vi "UnscentedKalmanFilter_SetXHat.vi"(10 "xHat":T1, 11 "in UnscentedKalmanFiilter":T2) -> (0 "SizeCoerced":bool, 3 "out UnscentedKalmanFiilter":T2)   [LabVIEW 2019, in "Trajectory_Library.lvlib"]
doc: "Set initial state estimate x-hat.\n \nInputs:\n - inUnscentedKalmanFilter -- filter data cluster\n - xHat -- The state estimate x-hat.\n\nOutputs:\n - outUnscentedKalmanFilter -- updated filter data cluster\n - sizeCoerced -- If TRUE, an error occured"
uses:
  Trajectory_Library.lvlib
  <vilib>/Analysis/Matrix/Datatypes/RealMatrix.ctl
  <vilib>/Analysis/Matrix/NI_Matrix.lvlib
  TypeDef/MERWE_SCALED_SIGMA_PTS.ctl
  TypeDef/UNSCENTED_KALMAN_FILTER.ctl
  TypeDef/CALLBACK_FUNC_TYPE.ctl
panel:
  # "State Estimate <Statess,1>"
  # "<States, States>"
  # "<States, ?>"
  # "<Statess,  States>"
  # "<Outputs, Outputs>"
  # "<?, 1>"
  # "<?, 1>"
  # "State Estimate <Statess,1>"
  # "<States, States>"
  # "<States, ?>"
  # "<Statess,  States>"
  # "<Outputs, Outputs>"
  # "<?, 1>"
  # "<?, 1>"
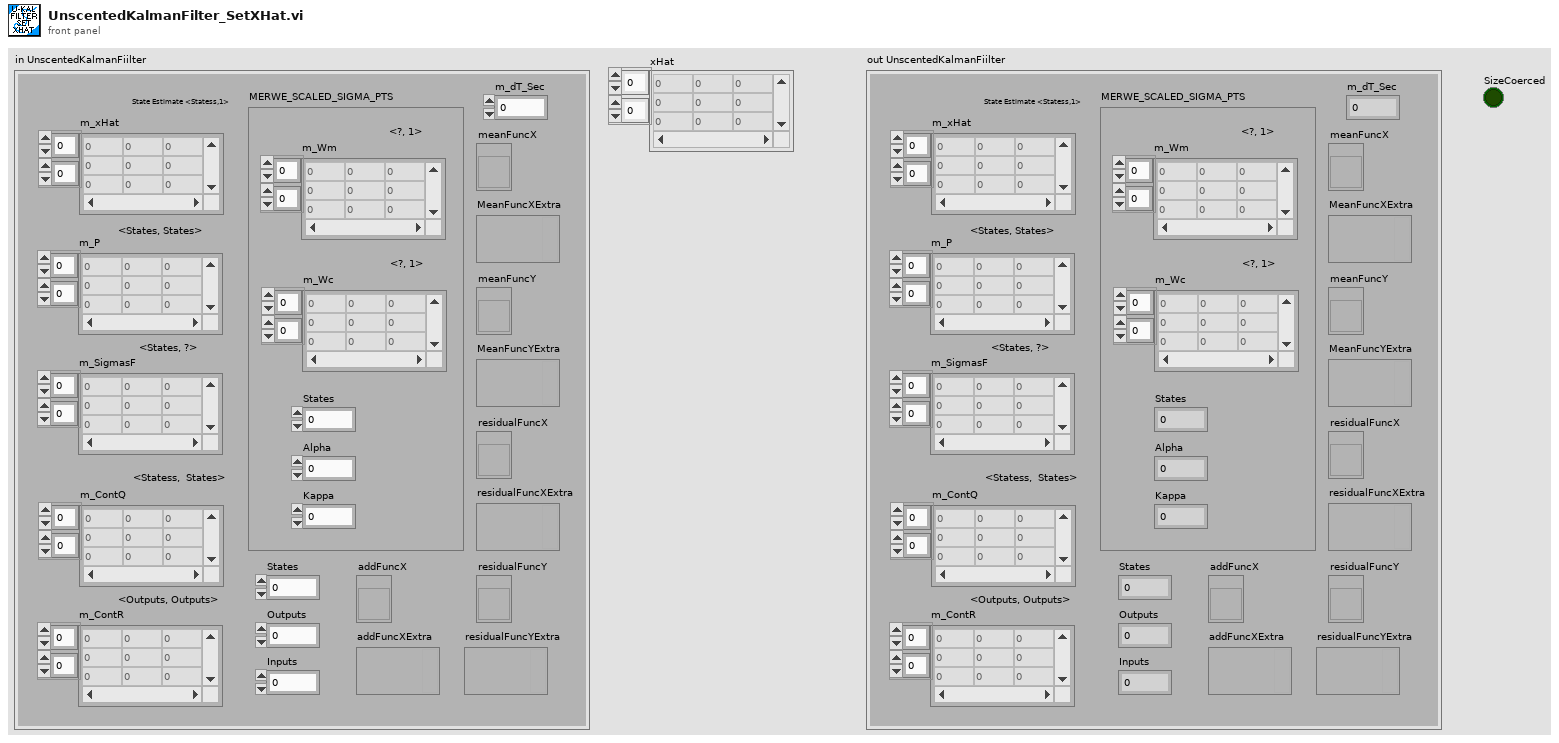
[diagram p1: front panel]
types:
  T1 = typedef "NI_Matrix.lvlib/RealMatrix.ctl" = dbl[][]
  T2 = typedef "Trajectory_Library.lvlib/UNSCENTED_KALMAN_FILTER.ctl" = cluster{"m_P":T1, "m_xHat":T1, "States":i32, "Outputs":i32, "m_ContR":T1, "m_ContQ":T1, "m_SigmasF":T1, "m_dT_Sec":dbl, "MERWE_SCALED_SIGMA_PTS":T3, "meanFuncX":T4, "meanFuncY":T4, "residualFuncX":T4, "residualFuncY":T4, "addFuncX":T4, "addFuncXExtra":variant, "residualFuncYExtra":variant, "residualFuncXExtra":variant, "MeanFuncYExtra":variant, "MeanFuncXExtra":variant, "Inputs":i32}
  T3 = typedef "Trajectory_Library.lvlib/MERWE_SCALED_SIGMA_PTS.ctl" = cluster{"m_Wm":T1, "States":i32, "Alpha":dbl, "m_Wc":T1, "Kappa":i32}
  T4 = typedef "Trajectory_Library.lvlib/CALLBACK_FUNC_TYPE.ctl" = refnum<vi>
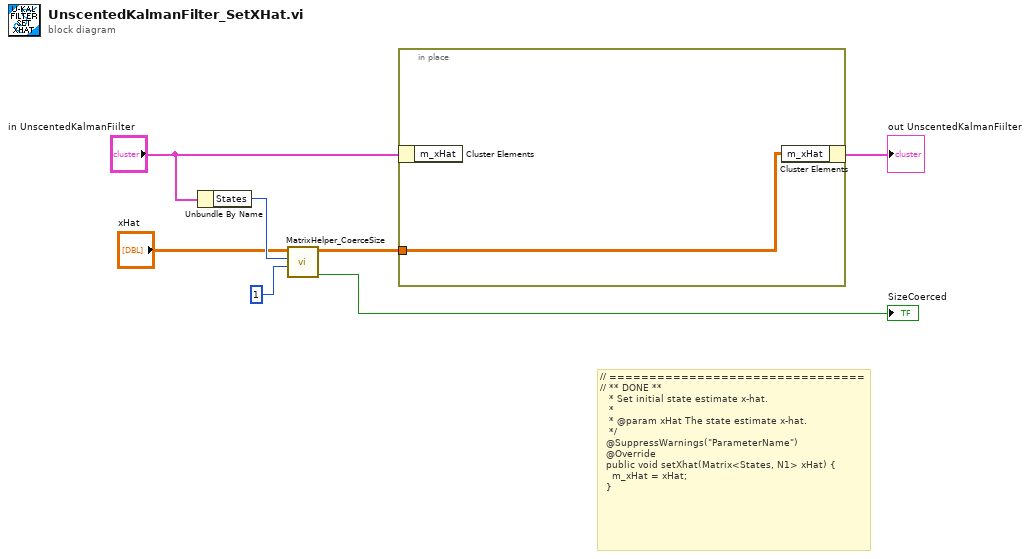
[diagram p0: block diagram]
diagram:
  # "// ================================\n// ** DONE **\n   * Set initial state estimate x-hat.\n   *\n   * @param xHat The state estimate x-hat.\n   */\n  @SuppressWarnings(\"ParameterName\")\n  @Override\n  public void setXhat(Matrix<States, N1> xHat) {\n    m_xHat = xHat;\n  }"
  n1 = Unbundle By Name("in UnscentedKalmanFiilter") -> ("States"=w6:i32)
  n2 = call "MatrixHelper_CoerceSize.vi"("Columns"=1, "Rows"=w6, "input matrix"="xHat") -> ("Coerced"=→"SizeCoerced":bool, "output matrix"=w3:T1)  [unwired: 7 in]
  n3 = in-place {
    in-place-border: w3 -> [w8]
    n4 = in-place-cluster #1("in UnscentedKalmanFiilter") -> ()  [unwired: 1 out]
    n5 = in-place-cluster #1("m_xHat"=w8) -> (→"out UnscentedKalmanFiilter":T2)
  }
